vi "Add Parameter.vi"(8 "error in":errorcluster, 9 "parameter encoding":T1={"start index"=0, "size"=8, "encoding"=enum."BCD", "signed"=FALSE, "scale multiplier"=1.0, "scale offset"=0.0, "default value"=0.0}, 10 "parameter definition":cluster{"name":string, "unit":string}, 11 "label ref":T3 format="%.0x") -> (0 "error out":errorcluster, 2 "parameter":T3 format="%.0x", 3 "label ref out":T3 format="%.0x")   [LabVIEW 2026, in "AIM ARINC 429 Scripting.lvlib"]
doc: "Adds the specified <b>parameter definition</b> with <b>parameter encoding</b> to the system definition in the 'Word' subsection of <b>label ref</b>. Returns the newly added <b>parameter</b> reference."
uses:
  AIM ARINC 429 Scripting.lvlib
  <vilib>/NI VeriStand/Custom Device API/Custom Device Item Ref.ctl
  Shared/Parameter Definition.ctl
  <vilib>/NI/NI VeriStand Encoding and Decoding/Encoding.ctl
  <vilib>/NI VeriStand/Custom Device API/Custom Device Channel.ctl
  <vilib>/NI VeriStand/Custom Device API/Custom Device Channel Type.ctl
  Constants.vi
  <vilib>/NI VeriStand/Custom Device API/Custom Device API.lvlib
  <vilib>/NI VeriStand/Custom Device Offline API/Custom Device Offline API.lvlib
  <vilib>/NI/NI VeriStand Encoding and Decoding/Encoding and Decoding.lvlib
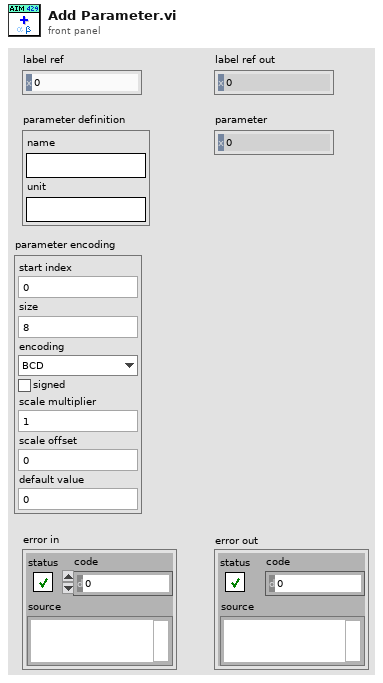
[diagram p1: front panel]
types:
  T1 = typedef "Parameter Definition.ctl" = cluster{"start index":i32, "size":i32, "encoding":T2, "signed":bool, "scale multiplier":dbl, "scale offset":dbl, "default value":dbl}
  T2 = typedef "Encoding and Decoding.lvlib/Encoding.ctl" = enum16{"BNR", "BCD", "Discrete"}
  T3 = typedef "Custom Device API.lvlib/Custom Device Item Ref.ctl" = u64
  T4 = typedef "Custom Device API.lvlib/Custom Device Channel.ctl" = cluster{"Type":T5, "Units":string, "Default Value":dbl, "Faultable":bool, "Scalable":bool}
  T5 = typedef "Custom Device API.lvlib/Custom Device Channel Type.ctl" = enum16{"Input", "Output"}
  T6 = typedef "Direction.ctl" = enum16{"Rx", "Tx"}
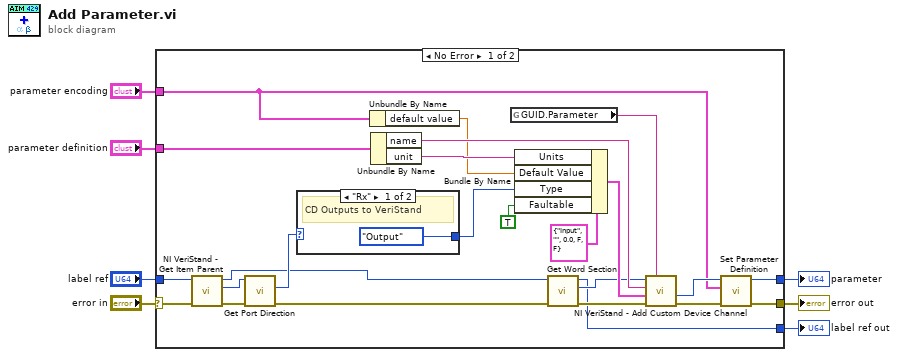
[diagram p0: block diagram]
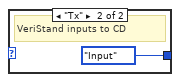
[diagram p2: hidden frame]
diagram:
  n1 = case shown="No Error" "error in" {
    selector: "error in" -> [w21 w35]
    tunnel: [w23 w35] -> w6
    tunnel: "label ref" -> [w20 w34]
    tunnel: [w24 _] -> w4
    tunnel: "parameter definition" -> [w27 _]
    tunnel: [w11 w34] -> w2
    tunnel: "parameter encoding" -> [w10 _]
    frame No Error {
      n2 = call <vilib>:"NI VeriStand - Get Item Parent.vi"("error in (no error)"=w21, "Item Ref in"=w20) -> ("error out"=w19:errorcluster, "Parent Ref"=w14:T3, "Item Ref out"=w13:T3)  [unwired: 6 in, 1 out]
      n3 = call "Get Port Direction.vi"("error in"=w19, "port ref"=w14) -> ("error out"=w18:errorcluster, "direction"=w17:T6)  [unwired: 7 in, 1 out]
      n4 = case shown="\"Rx\"" w17 {
        tunnel: [Custom_Device_Channel_Type."Output" ("Type") Custom_Device_Channel_Type."Input" ("Type")] -> w16
        frame "Rx" {
          # "CD Outputs to VeriStand"
        }
        frame "Tx" {
          # "VeriStand inputs to CD"
        }
      }
      n5 = Unbundle By Name(w10) -> ("default value"=w9:dbl)
      n6 = Unbundle By Name(w27) -> ("name"=w15:string, "unit"=w28:string)
      n7 = global read "Constants.vi" "GUID.Parameter"() -> (w31:string)
      n8 = Bundle By Name(cluster=T4 {"Type"=enum."Input", "Units"="", "Default Value"=0.0, "Faultable"=FALSE, "Scalable"=FALSE} ("Channel"), "Units"=w28, "Default Value"=w9, "Type"=w16, "Faultable"=TRUE) -> (w29:T4)
      n9 = call "Get Word Section.vi"("error in"=w18, "label ref"=w13) -> ("error out"=w22:errorcluster, "word ref"=w12:T3, "label ref out"=w11:T3)  [unwired: 7 in]
      n10 = call <vilib>:"NI VeriStand - Add Custom Device Channel.vi"("GUID (Default Channel)"=w31, "error in (no error)"=w22, "Channel"=w29, "Channel Name"=w15, "Parent Ref in"=w12) -> ("error out"=w26:errorcluster, "Channel Ref"=w25:T3)  [unwired: 3 in, 2 out]
      n11 = call "Set Parameter Definition.vi"("error in"=w26, "parameter definition"=w10, "parameter ref"=w25) -> ("error out"=w23:errorcluster, "parameter ref out"=w24:T3)  [unwired: 7 in]
    }
    frame Error {
    }
  }
  "parameter" <- w4
  "error out" <- w6
  "label ref out" <- w2
